vi "Bezier Trajectory.vi"(5 "Turn Rate":dbl=5.0 format="%#_13g", 6 "Overrides":T1 {"Angle Override" step=5.0; "Velocity Override" step=5.0; "Angular Override" step=5.0}, 7 "Drive Type":T4, 8 "Conditions":T7, 9 "All Limits":cluster{"Limits":T2, "Angular Limits":T3} {"Limits"."StoopidFast (fps)" min=0.0; "Limits"."Jerk (fps^3)" min=0.0 step=1.0; "Limits"."Accel (fps^2)" min=0.0; "Limits"."Velocity (fps)" min=0.0; "Angular Limits"."Jerk (deg/s^3)" min=0.0 step=1.0; "Angular Limits"."Accel (deg/s^2)" min=0.0; "Angular Limits"."Velocity (deg/s)" min=0.0}, 10 "sample period (s)":sgl, 11 "WayPoints":T8) -> (0 "Time & Dist":cluster{"Time (s)":dbl, "Distance (ft)":dbl}, 1 "Valid":bool, 2 "Updated Waypoints":cluster{"x":dbl, "y":dbl, "th":dbl}[](array[cluster]), 3 "Trajectory Data":T5)   [LabVIEW 2023]
uses:
  Types/Waypoints.ctl
  Types/Trajectory Data.ctl
  Types/Segment Type.ctl
  Types/Drive Type.ctl
  Types/Limits.ctl
  Types/Angluar Limits.ctl
  Types/Overrides.ctl
panel:
  out "XY Graph":cluster{"X":dbl, "Y":dbl}[](graph)
  in  "dynamic?":bool
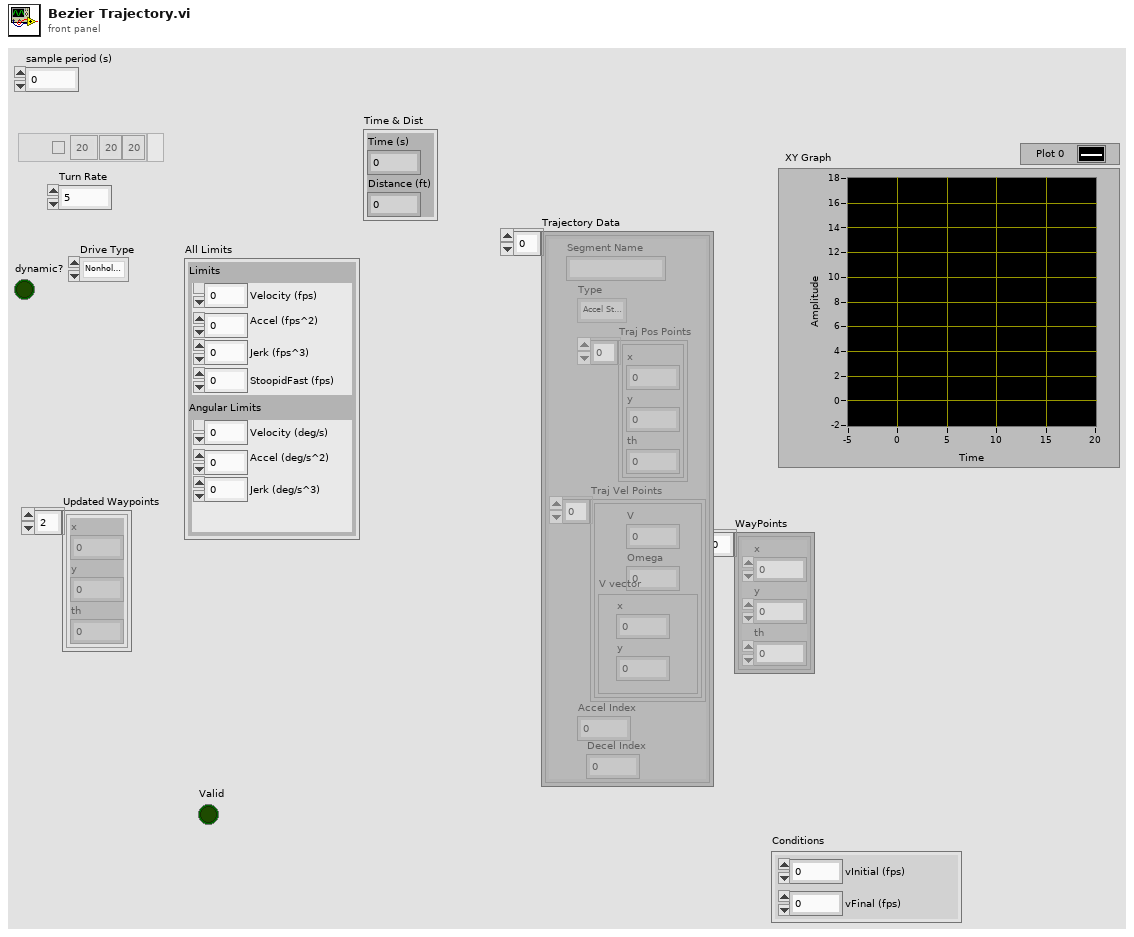
[diagram p1: front panel]
types:
  T1 = typedef "Overrides.ctl" = cluster{"Count":string, "Angular Override":dbl, "Enabled?":bool, "Velocity Override":dbl, "Angle Override":dbl}[]
  T2 = typedef "Limits.ctl" = cluster{"Velocity (fps)":dbl, "Accel (fps^2)":dbl, "Jerk (fps^3)":dbl, "StoopidFast (fps)":dbl}
  T3 = typedef "Angluar Limits.ctl" = cluster{"Velocity (deg/s)":dbl, "Accel (deg/s^2)":dbl, "Jerk (deg/s^3)":dbl}
  T4 = typedef "Drive Type.ctl" = enum16{"Nonholonomic", "Holonomic"}
  T5 = typedef "Trajectory Data.ctl" = cluster{"Segment Name":string, "Type":T6, "Traj Pos Points":cluster{"x":dbl, "y":dbl, "th":dbl}[], "Traj Vel Points":cluster{"V":dbl, "Omega":dbl, "V vector":cluster{"y":dbl, "x":dbl}}[], "Accel Index":i32, "Decel Index":i32}[]
  T6 = typedef "Segment Type.ctl" = enum16{"Accel Straight", "Const Straight", "Blend", "Circle", "Bezier"}
  T7 = cluster{"vInitial (fps)":dbl, "vFinal (fps)":dbl}
  T8 = typedef "Waypoints.ctl" = cluster{"x":sgl, "y":sgl, "th":sgl}[]
  T9 = cluster{"Velocity (fps)":dbl, "Accel (fps^2)":dbl, "Jerk (fps^3)":dbl}
  T10 = typedef "Bezier Curve.ctl" = cluster{"x":sgl, "y":sgl}[]
  T11 = cluster{"Segment Name":string, "Type":T6, "Traj Pos Points":cluster{"x":dbl, "y":dbl, "th":dbl}[], "Traj Vel Points":cluster{"V":dbl, "Omega":dbl, "V vector":cluster{"y":dbl, "x":dbl}}[], "Accel Index":i32, "Decel Index":i32}
  T12 = cluster{"Segment Name":string, "Type":T6, "Traj Pos Points":cluster{"x":dbl, "y":dbl, "th":dbl}[], "Traj Vel Points":cluster{"V":dbl, "Omega":dbl, "V vector":cluster{"y":dbl, "x":dbl}}[], "Accel Index":i32, "Decel Index":i32}[]
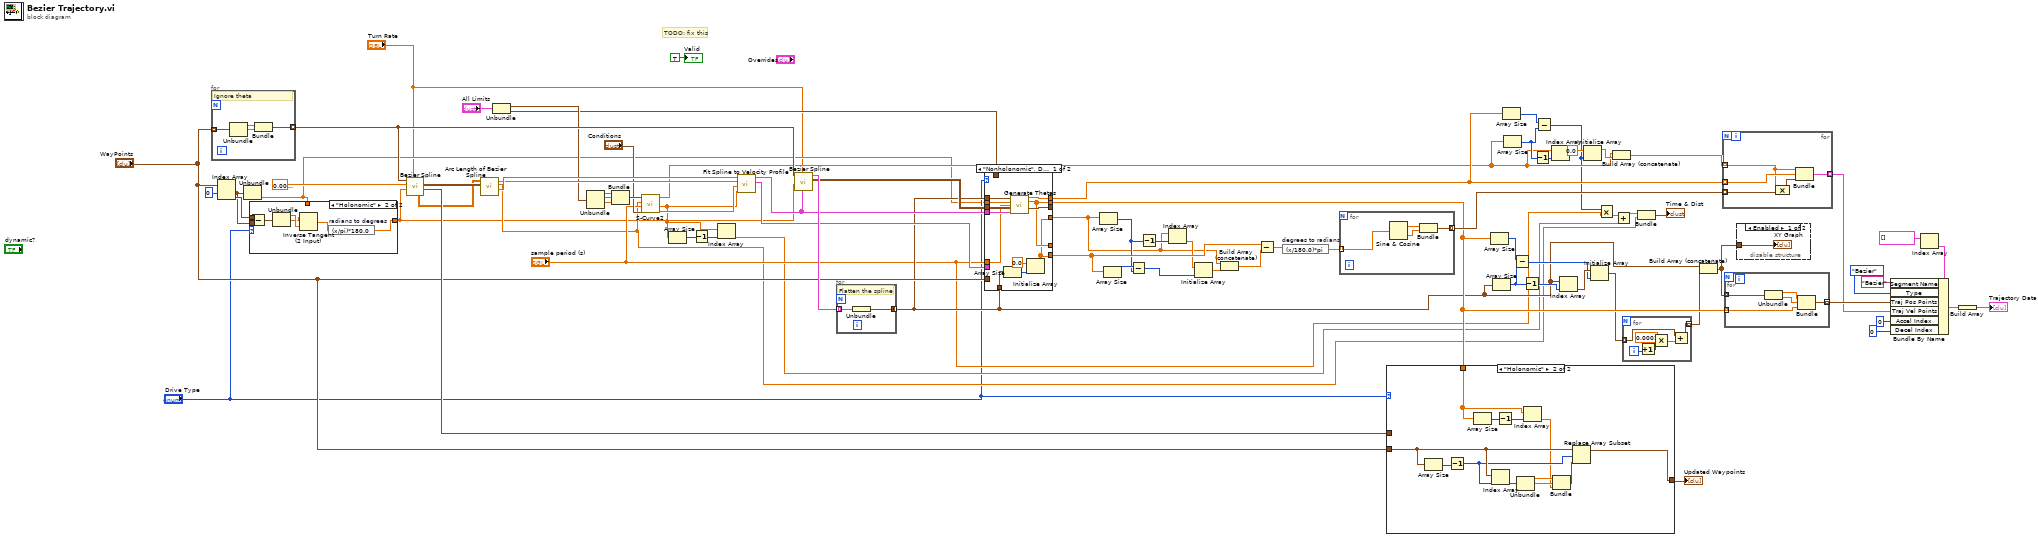
[diagram p0: block diagram]
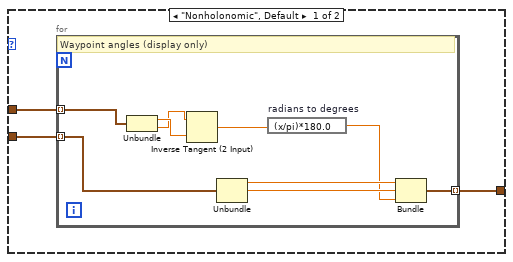
[diagram p4: hidden frame]
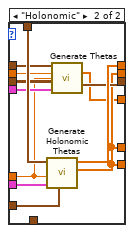
[diagram p5: hidden frame]
diagram:
  # "TODO: fix this"
  n1 = for {
    tunnel: "WayPoints" -> [w84] mode=indexing
    tunnel: [w81] -> w62 mode=indexing
    # "Ignore theta"
    n2 = Unbundle(w84) -> ("x"=w83:sgl, "y"=w82:sgl)  [unwired: 1 out]
    n3 = Bundle("x"=w83, "y"=w82) -> (w81:cluster{"x":sgl, "y":sgl})  [unwired: 1 in]
  }
  n4 = Index Array(array="WayPoints", index #1=0 ("index")) -> (element #1=w5:cluster{"x":sgl, "y":sgl, "th":sgl}, element #2=w6:cluster{"x":sgl, "y":sgl, "th":sgl})  [unwired: 1 in]
  n5 = Unbundle(w5) -> ("th"=w3:sgl)  [unwired: 2 out]
  n6 = case shown="\"Holonomic\"" "Drive Type" {
    tunnel: w6 -> [_ w92]
    tunnel: w5 -> [_ w91]
    tunnel: [w85 w86] -> w2
    tunnel: w3 -> [w85 _]
    frame "Nonholonomic", Default {
    }
    frame "Holonomic" {
      n7 = Subtract(x=w92, y=w91) -> (x-y=w90:cluster{"x":sgl, "y":sgl, "th":sgl})
      n8 = Unbundle(w90) -> ("x"=w89:sgl, "y"=w88:sgl)  [unwired: 1 out]
      n9 = Inverse Tangent (2 Input)(1:w89, 2:w88) -> (0:w87:sgl)
      n10 = expression code="(x/pi)*180.0" "radians to degrees"(w87) -> (w86:sgl)
    }
  }
  n11 = call "Bezier Spline.vi"("Turn Rate"="Turn Rate", "starting orientation (deg)"=w2, "percision"=sgl 0.01, "waypts"=w62) -> ("Tangents"=w75:cluster{sgl, sgl}[], "ctrl pts"=w65:cluster{sgl, sgl}[][], "position out"=w59:sgl[][])  [unwired: 3 in, 2 out]
  n12 = call "Arc Length of Bezier Spline.vi"("ctrl pts"=w65, "position"=w59) -> ("t"=w64:sgl[], "l total"=w9:dbl, "l"=w63:dbl[])  [unwired: 6 in, 1 out]
  n13 = Unbundle("All Limits") -> ("Limits"=w52:T2, "Angular Limits"=w51:T3)
  n14 = Unbundle(w52) -> ("Velocity (fps)"=w79:dbl, "Accel (fps^2)"=w78:dbl, "Jerk (fps^3)"=w77:dbl)  [unwired: 1 out]
  n15 = Bundle("Velocity (fps)"=w79, "Accel (fps^2)"=w78, "Jerk (fps^3)"=w77) -> (w76:T9)  [unwired: 1 in]
  n16 = call "S-Curve2.vi"("Conditions"="Conditions", "dt (s)"="sample period (s)", "goal"=w9, "Limits"=w76) -> ("X"=w61:dbl[], "T"=w55:dbl[], "V"=w19:dbl[])  [unwired: 5 in]
  n17 = Array Size(array=w55) -> (size(s)=w74:i32)
  n18 = Decrement(x=w74) -> (x-1=w73:i32)
  n19 = Index Array(array=w55, index=w73) -> (element=w10:dbl)
  n20 = call "Fit Spline to Velocity Profile.vi"("time"=w55, "vel positions"=w61, "s(t)"=w63, "t flat"=w64) -> ("time unflat"=w54:cluster{dbl[]}[], "y unflat"=w56:cluster{dbl[]}[])  [unwired: 6 in]
  n21 = call "Bezier Spline.vi"("positions"=w56, "Turn Rate"="Turn Rate", "starting orientation (deg)"=w2, "waypts"=w62) -> ("ctrl pts"=w57:cluster{sgl, sgl}[][], "bezier spline"=w58:cluster{"curve ":T10}[])  [unwired: 3 in, 3 out]
  n22 = for {
    tunnel: w58 -> [w94] mode=indexing
    tunnel: [w93] -> w35 mode=concatenating
    # "Flatten the spline"
    n23 = Unbundle(w94) -> ("curve"=w93:T10)
  }
  n24 = case shown="\"Nonholonomic\", Default" "Drive Type" {
    tunnel: [w106 w118] -> w25
    tunnel: [w100 w109] -> w41
    tunnel: w3 -> [w105 w113]
    tunnel: w35 -> [w104 w114]
    tunnel: w57 -> [w103 w112]
    tunnel: w56 -> [w102 w111]
    tunnel: w54 -> [_ w117]
    tunnel: "sample period (s)" -> [w95 w107]
    tunnel: w51 -> [_ w116]
    tunnel: "WayPoints" -> [_ w115]
    tunnel: [w101 w110] -> _
    tunnel: [w100 w109] -> _
    tunnel: [w96 w109] -> w34
    tunnel: [w96 w108] -> w28
    tunnel: w35 -> [w99 _]
    frame "Nonholonomic", Default {
      n25 = Array Size(array=w99) -> (size(s)=w98:i32)
      n26 = call "Generate Thetas.vi"("spline flat"=w104, "starting angle"=w105, "dt"=w95, "ctrl pts"=w103, "y unflat"=w102) -> ("omega"=w106:sgl[], "theta"=w100:sgl[], "Tangent Vector"=w101:cluster{"x out":dbl, "y out":dbl}[])  [unwired: 8 in]
      n27 = Initialize Array(0.0 ("element"), w98) -> (w96:dbl[])
    }
    frame "Holonomic" {
      n28 = call "Generate Holonomic Thetas.vi"("WayPoints"=w115, "time unflat"=w117, "dt"=w107, "Angular Limits"=w116) -> ("X"=w109:dbl[], "V"=w118:dbl[])  [unwired: 6 in]
      n29 = call "Generate Thetas.vi"("spline flat"=w114, "starting angle"=w113, "dt"=w107, "ctrl pts"=w112, "y unflat"=w111) -> ("theta"=w108:sgl[], "Tangent Vector"=w110:cluster{"x out":dbl, "y out":dbl}[])  [unwired: 8 in, 1 out]
    }
  }
  n30 = Array Size(array=w28) -> (size(s)=w31:i32)
  n31 = Array Size(array=w34) -> (size(s)=w33:i32)
  n32 = Subtract(x=w33, y=w31) -> (x-y=w32:i32)
  n33 = Decrement(x=w31) -> (x-1=w30:i32)
  n34 = Index Array(array=w28, index=w30) -> (element=w29:dbl)
  n35 = Initialize Array(w29, w32) -> (w27:dbl[])
  n36 = Build Array (concatenate)(w28, w27) -> (w26:dbl[])
  n37 = Subtract(x=w34, y=w26) -> (x-y=w42:dbl[])
  n38 = expression code="(x/180.0)*pi" "degrees to radians"(w42) -> (w43:dbl[])
  n39 = for {
    tunnel: w43 -> [w120] mode=indexing
    tunnel: [w122] -> w44 mode=indexing
    n40 = Sine & Cosine(0:w120) -> (1:w121:dbl, 2:w119:dbl)
    n41 = Bundle(w121, w119) -> (w122:cluster{dbl, dbl})  [unwired: 1 in]
  }
  n42 = case shown="\"Holonomic\"" "Drive Type" {
    tunnel: w75 -> [w125 _]
    tunnel: "WayPoints" -> [w124 w142]
    tunnel: [w123 w135] -> w50
    tunnel: w41 -> [_ w144]
    frame "Nonholonomic", Default {
      n43 = for {
        tunnel: w124 -> [w134] mode=indexing
        tunnel: w125 -> [w126] mode=indexing
        tunnel: [w131] -> w123 mode=indexing
        # "Waypoint angles (display only)"
        n44 = Unbundle(w126) -> (w129:sgl, w128:sgl)
        n45 = Inverse Tangent (2 Input)(1:w129, 2:w128) -> (0:w127:sgl)
        n46 = Unbundle(w134) -> ("x"=w133:sgl, "y"=w132:sgl)  [unwired: 1 out]
        n47 = expression code="(x/pi)*180.0" "radians to degrees"(w127) -> (w130:sgl)
        n48 = Bundle("x"=w133, "y"=w132, w130) -> (w131:cluster{"x":sgl, "y":sgl, sgl})  [unwired: 1 in]
      }
    }
    frame "Holonomic" {
      n49 = Array Size(array=w142) -> (size(s)=w143:i32)
      n50 = Decrement(x=w143) -> (x-1=w141:i32)
      n51 = Array Size(array=w144) -> (size(s)=w146:i32)
      n52 = Index Array(array=w142, index=w141) -> (element=w140:cluster{"x":sgl, "y":sgl, "th":sgl})
      n53 = Decrement(x=w146) -> (x-1=w145:i32)
      n54 = Unbundle(w140) -> ("x"=w139:sgl, "y"=w138:sgl)  [unwired: 1 out]
      n55 = Index Array(array=w144, index=w145) -> (element=w137:dbl)
      n56 = Bundle("x"=w139, "y"=w138, w137) -> (w136:cluster{"x":sgl, "y":sgl, dbl})  [unwired: 1 in]
      n57 = Replace Array Subset(array=w142, new element=w136, index=w141) -> (w135:T8)
    }
  }
  "Updated Waypoints" <- w50
  n58 = Array Size(array=w41) -> (size(s)=w40:i32)
  n59 = Array Size(array=w35) -> (size(s)=w39:i32)
  n60 = Array Size(array=w25) -> (size(s)=w24:i32)
  n61 = Array Size(array=w19) -> (size(s)=w23:i32)
  n62 = Subtract(x=w40, y=w39) -> (x-y=w36:i32)
  n63 = Decrement(x=w39) -> (x-1=w38:i32)
  n64 = Decrement(x=w23) -> (x-1=w22:i32)
  n65 = Subtract(x=w24, y=w23) -> (x-y=w15:i32)
  n66 = Index Array(array=w19, index=w22) -> ()  [unwired: 1 out]
  n67 = Index Array(array=w35, index=w38) -> (element=w37:cluster{"x":sgl, "y":sgl})
  n68 = Initialize Array(0.0 ("element"), w15) -> (w21:dbl[])
  n69 = Initialize Array(w37, w36) -> (w17:cluster{"x":sgl, "y":sgl}[])
  n70 = Multiply(x=w15, y="sample period (s)") -> (x*y=w14:sgl)
  n71 = Build Array (concatenate)(w19, w21) -> (w18:dbl[])
  n72 = Add(x=w14, y=w10) -> (x+y=w13:dbl)
  n73 = for {
    tunnel: w17 -> [w148] mode=indexing
    tunnel: [w147] -> w16 mode=indexing
    i -> [w151]
    n74 = Increment(x=w151) -> (x+1=w150:i32)
    n75 = Multiply(x=0.0001, y=w150) -> (x*y=w149:dbl)
    n76 = Add(x=w148, y=w149) -> (x+y=w147:cluster{"x":dbl, "y":dbl})
  }
  n77 = Bundle(w13, "l total"=w9) -> (→"Time & Dist":cluster{dbl, "l total":dbl})  [unwired: 1 in]
  n78 = Build Array (concatenate)(w35, w16) -> (w8:cluster{"x":dbl, "y":dbl}[])
  n79 = for {
    tunnel: w25 -> [w157] mode=indexing
    tunnel: w18 -> [w153] mode=indexing
    tunnel: [w156] -> w68 mode=indexing
    tunnel: w44 -> [w154] mode=indexing
    n80 = Compound Arithmetic op=MULTIPLY(w153, w154) -> (w155:cluster{dbl, dbl})
    n81 = Bundle("element"=w153, w157, w155) -> (w156:cluster{"element":dbl, dbl, cluster{dbl, dbl}})  [unwired: 1 in]
  }
  n82 = for {
    tunnel: w8 -> [w162] mode=indexing
    tunnel: [w159] -> w69 mode=indexing
    tunnel: w41 -> [w158] mode=indexing
    n83 = Unbundle(w162) -> ("x"=w161:dbl, "y"=w160:dbl)
    n84 = Bundle("x"=w161, "y"=w160, w158) -> (w159:cluster{"x":dbl, "y":dbl, dbl})  [unwired: 1 in]
  }
  n85 = disable-structure shown="Enabled" {
    disable-tunnel: w8 -> [w163 _]
    frame Enabled {
      "XY Graph" <- w163
    }
    frame Disabled {
    }
  }
  n86 = Index Array(array=T5 [] ("Trajectory Data")) -> (element=w45:T11)  [unwired: 1 in]
  n87 = Bundle By Name(cluster=w45, "Segment Name"="Bezier", "Type"=Segment_Type."Bezier", "Traj Pos Points"=w69, "Traj Vel Points"=w68, "Accel Index"=0, "Decel Index"=0) -> (w7:T11)
  n88 = Build Array(w7) -> (→"Trajectory Data":T12)
  "Valid" <- TRUE ("Valid")
